vi "Read Comm to Main.vi"(8 "error in (no error)":errorcluster, 11 "CIFPlugin in":refnum<class "CAN_Writer_NIXNET_Plugin.lvclass">) -> (0 "error out":errorcluster, 3 "CIFPlugin out":refnum<class "CAN_Writer_NIXNET_Plugin.lvclass">)   [LabVIEW 2021, in "CAN_Writer_NIXNET_Plugin.lvclass"]
uses:
  CAN_Writer_NIXNET_Plugin.lvclass
  CAN_Writer_NIXNET_Plugin.lvclass/CAN_Writer_NIXNET_Plugin.ctl
  525c214c-2a6b-4e7b-b3ce-0ad96b412d2f.vi
  Common/Typedef/OOB Comm/To Main Command.ctl
  Common/CAN_Writer_NIXNET_Common.lvlib
  Common/Typedef/OOB Comm/To Main Command Data.ctl
  Common/Typedef/OOB Comm/To Main Command Payload.ctl
  4efb0375-f1de-4191-b03f-44d34e6646cb.vi
  <vilib>/CIF Foundation/CIF CIPC/TypeDefs/Read Position.ctl
  <vilib>/CIF Foundation/CIF CIPC/CIF_NI_CIPC.lvlib
  <vilib>/CIF Foundation/CIF CIPC/TypeDefs/Read Configuration.ctl
  <vilib>/CIF Foundation/CIF XNET CAN RW/XNET CAN RW.lvclass
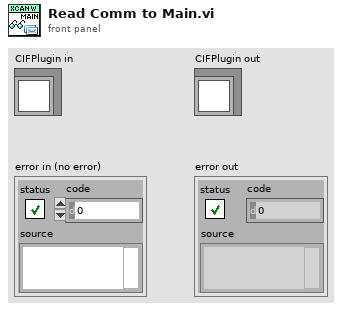
[diagram p1: front panel]
types:
  T1 = typedef "CIF_NI_CIPC.lvlib/Read Configuration.ctl" = cluster{"Read Position":T2, "Element Offset":i32, "Prepend Array Size":bool, "Get Read Position":bool}
  T2 = typedef "CIF_NI_CIPC.lvlib/Read Position.ctl" = enum8{"Next", "Newest", "Oldest", "Next Available", "Absolute"}
  T3 = typedef "CAN_Writer_NIXNET_Common.lvlib/To Main Command Payload.ctl" = cluster{"Command":T4, "-> Main":T5}
  T4 = typedef "CAN_Writer_NIXNET_Common.lvlib/To Main Command.ctl" = enum16{"Read Data", "Read DVR Data", "Output Message"}
  T5 = typedef "CAN_Writer_NIXNET_Common.lvlib/To Main Command Data.ctl" = cluster{"Cmd Data 1 -> Main":i32}
  T6 = typedef "CAN_Writer_NIXNET_Common.lvlib/To Main DVR Data.ctl" = cluster{"Data 1 DVR  -> Main":i32, "Output Message":u8[]}
  T7 = typedef "CIFCorePlugin.lvclass/Energized States.ctl" = enum8{"Listen", "Prepare", "Execute", "Housekeep", "Cleanup", "Destroy"}
  T8 = typedef "CAN_Writer_NIXNET_Common.lvlib/To Main Cyclic Data.ctl" = cluster{"Data 1 -> Main":i32}
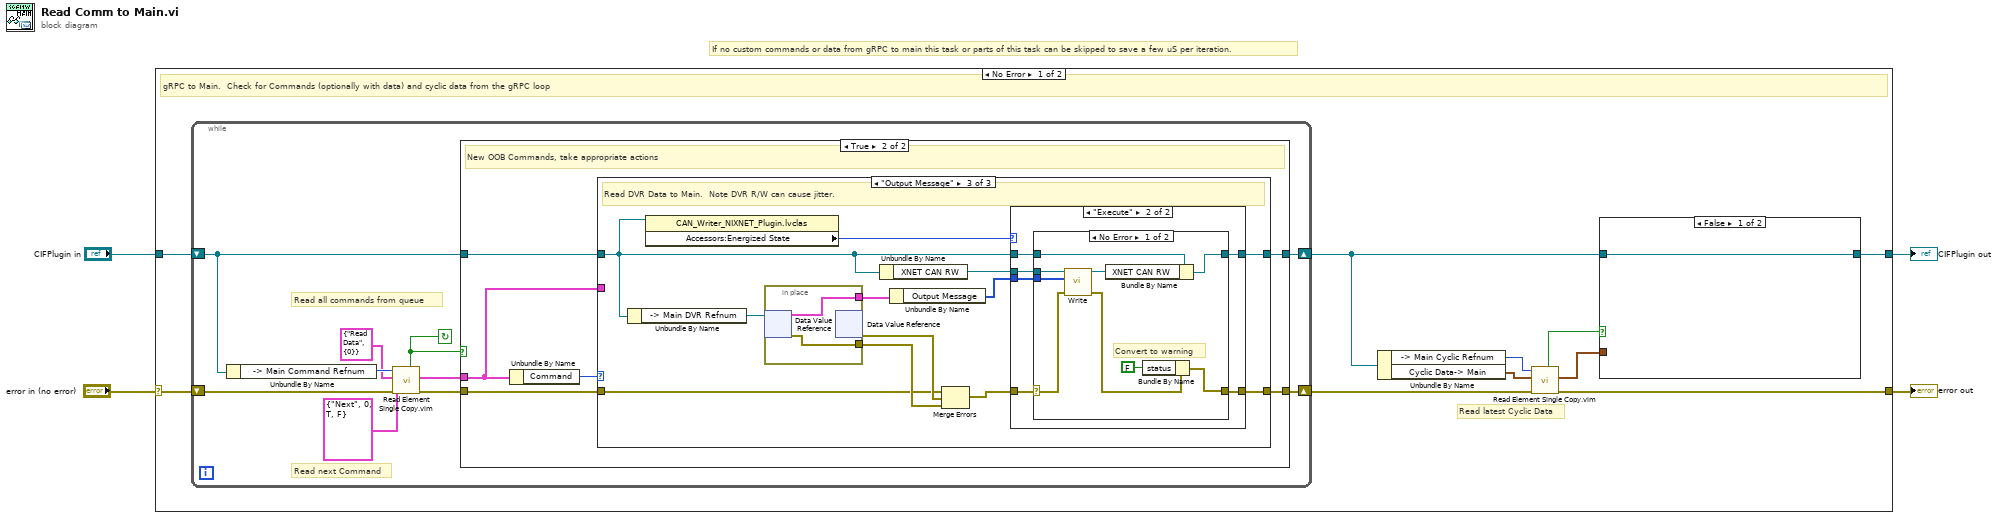
[diagram p0: block diagram]
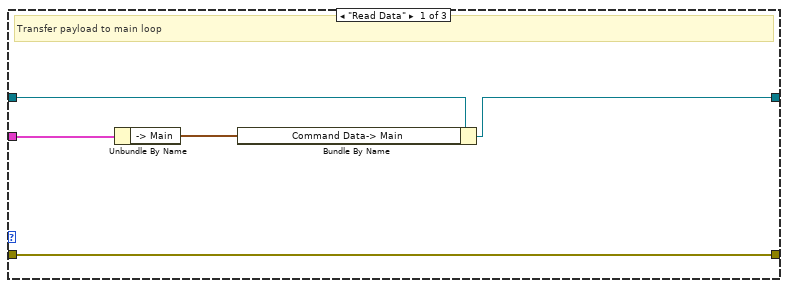
[diagram p3: hidden frame]
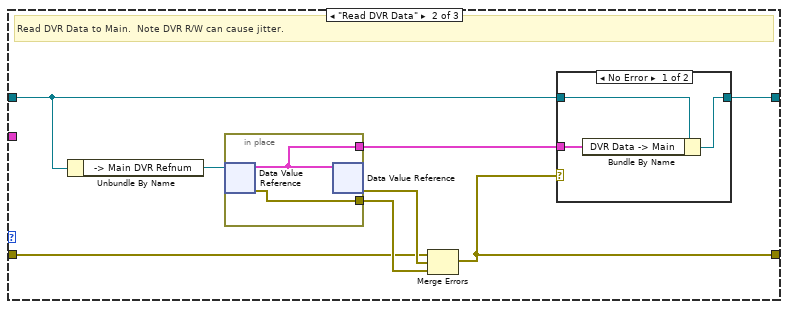
[diagram p4: hidden frame]
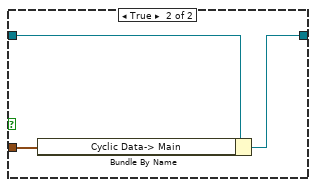
[diagram p8: hidden frame]
diagram:
  # "If no custom commands or data from gRPC to main this task or parts of this task can be skipped to save a few uS per iteration."
  n1 = case shown="No Error" "error in (no error)" {
    selector: "error in (no error)" -> [w14 w90]
    tunnel: [w10 w90] -> w3
    tunnel: [w5 w89] -> w1
    tunnel: "CIFPlugin in" -> [w13 w89]
    frame No Error {
      # "Read latest Cyclic Data"
      # "gRPC to Main.  Check for Commands (optionally with data) and cyclic data from the gRPC loop"
      n2 = while {
        shift-right: [w19] -> w11
        shift-left: w14 -> [w23]
        shift-right: [w17] -> w6
        shift-left: w13 -> [w15]
        stop <- w16 continue-if-true
        # "Read all commands from queue"
        # "Read next Command"
        n3 = Unbundle By Name(w15) -> ("-> Main Command Refnum"=w24:u64)
        n4 = call "Read Element Single Copy.vim"("error in (no error)"=w23, "Read Configuration"=T1 {"Read Position"=enum."Next", "Element Offset"=0, "Prepend Array Size"=TRUE, "Get Read Position"=FALSE}, "Data in"=T3 {"Command"=enum."Read Data", "-> Main"={"Cmd Data 1 -> Main"=0}} ("Payload"), "CIPC Reference in"=w24) -> ("error out"=w21:errorcluster, "Data out"=w20:T3, "Success"=w16:bool)  [unwired: 3 in, 2 out]
        n5 = case shown="True" w16 {
          tunnel: w15 -> [w26 w32]
          tunnel: [w26 w27] -> w17
          tunnel: w21 -> [w25 w31]
          tunnel: [w25 w30] -> w19
          tunnel: w20 -> [_ w28]
          frame False {
            # "No new OOB Commands"
          }
          frame True {
            # "New OOB Commands, take appropriate actions"
            n6 = Unbundle By Name(w28) -> ("Command"=w29:T4)
            n7 = case shown="\"Output Message\"" w29 {
              tunnel: w31 -> [w37 w41 w60]
              tunnel: w32 -> [w35 w40 w54]
              tunnel: [w37 w38 w55] -> w30
              tunnel: w28 -> [w36 _ _]
              tunnel: [w33 w39 w59] -> w27
              frame "Read Data" {
                # "Transfer payload to main loop"
                n8 = Unbundle By Name(w36) -> ("-> Main"=w34:T5)
                n9 = Bundle By Name(cluster=w35, "Command Data-> Main"=w34) -> (w33:refnum<class "CAN_Writer_NIXNET_Plugin.lvclass">)
              }
              frame "Read DVR Data" {
                # "Read DVR Data to Main.  Note DVR R/W can cause jitter."
                n10 = Unbundle By Name(w40) -> ("-> Main DVR Refnum"=w43:refnum<data-value>)
                n11 = in-place {
                  in-place-border: [w51] -> w45
                  in-place-border: [w50] -> w42
                  n12 = in-place-dvr #1(w43) -> (w50:T6, w51:errorcluster)
                  n13 = in-place-dvr #1(w50) -> (w44:errorcluster)  [unwired: 1 out]
                }
                n14 = Merge Errors(w41, w44, w45) -> (w38:errorcluster)
                n15 = case shown="No Error" w38 {
                  tunnel: w42 -> [w48 _]
                  tunnel: w40 -> [w47 w49]
                  tunnel: [w46 w49] -> w39
                  frame No Error {
                    n16 = Bundle By Name(cluster=w47, "DVR Data -> Main"=w48) -> (w46:refnum<class "CAN_Writer_NIXNET_Plugin.lvclass">)
                  }
                  frame Error {
                  }
                }
              }
              frame "Output Message" {
                # "Read DVR Data to Main.  Note DVR R/W can cause jitter."
                n17 = Unbundle By Name(w54) -> ("-> Main DVR Refnum"=w61:refnum<data-value>)
                n18 = property class="CAN_Writer_NIXNET_Plugin.lvclas"(reference=w54) -> ("Accessors:Energized State"=w52:T7)  [unwired: 1 in, 2 out]
                n19 = in-place {
                  in-place-border: [w84] -> w63
                  in-place-border: [w83] -> w58
                  n20 = in-place-dvr #2(w61) -> (w83:T6, w84:errorcluster)
                  n21 = in-place-dvr #2() -> (w62:errorcluster)  [unwired: 1 in, 1 out]
                }
                n22 = Unbundle By Name(w54) -> ("XNET CAN RW"=w57:refnum<class "XNET CAN RW.lvclass">)
                n23 = Unbundle By Name(w58) -> ("Output Message"=w53:u8[])
                n24 = Merge Errors(w60, w62, w63) -> (w56:errorcluster)
                n25 = case shown="\"Execute\"" w52 {
                  tunnel: [w65 w71] -> w59
                  tunnel: w57 -> [_ w70]
                  tunnel: w56 -> [w64 w69]
                  tunnel: [w64 w68] -> w55
                  tunnel: w54 -> [w65 w67]
                  tunnel: w53 -> [_ w66]
                  frame "Listen", Default {
                  }
                  frame "Execute" {
                    n26 = case shown="No Error" w69 {
                      selector: w69 -> [w75 w81]
                      tunnel: w67 -> [w80 w82]
                      tunnel: [w79 w82] -> w71
                      tunnel: w70 -> [w78 _]
                      tunnel: w66 -> [w77 _]
                      tunnel: [w72 w81] -> w68
                      frame No Error {
                        # "Convert to warning"
                        n27 = call-dynamic "Write.vi"("error in (no error)"=w75, "pcap CAN DATA in"=w77, "XNET_CAN_RW in"=w78) -> ("error out"=w74:errorcluster, "XNET_CAN_RW out"=w76:refnum<class "XNET CAN RW.lvclass">)  [unwired: 6 in, 1 out]
                        n28 = Bundle By Name(cluster=w80, "XNET CAN RW"=w76) -> (w79:refnum<class "CAN_Writer_NIXNET_Plugin.lvclass">)
                        n29 = Bundle By Name(cluster=w74, "status"=FALSE) -> (w72:errorcluster)
                      }
                      frame Error {
                      }
                    }
                  }
                }
              }
            }
          }
        }
      }
      n30 = Unbundle By Name(w6) -> ("-> Main Cyclic Refnum"=w12:u64, "Cyclic Data-> Main"=w9:T8)
      n31 = call "Read Element Single Copy.vim"("error in (no error)"=w11, "Data in"=w9, "CIPC Reference in"=w12) -> ("error out"=w10:errorcluster, "Data out"=w7:T8, "Success"=w8:bool)  [unwired: 4 in, 2 out]
      n32 = case shown="False" w8 {
        tunnel: w7 -> [_ w87]
        tunnel: w6 -> [w85 w88]
        tunnel: [w85 w86] -> w5
        frame False {
        }
        frame True {
          n33 = Bundle By Name(cluster=w88, "Cyclic Data-> Main"=w87) -> (w86:refnum<class "CAN_Writer_NIXNET_Plugin.lvclass">)
        }
      }
    }
    frame Error {
    }
  }
  "error out" <- w3
  "CIFPlugin out" <- w1
